vi "PathPlanner_TrajectoryState_Interpolate.vi"(9 "Time":dbl, 10 "end Val":T1={"TimeSeconds"=0.0, "VelocityMPS"=0.0, "AccerationMpsSq"=0.0, "HeadingAngularVelRadPerSec"=0.0, "PositionMeters"={"X"=0.0, "Y"=1.0}, "Heading"={"VALUE"=0.0, "COS"=1.0, "SIN"=0.0}, "TargetHolonomicRotation"={"VALUE"=0.0, "COS"=1.0, "SIN"=0.0}, "CurvatureRadPerMeter"=0.0, "PathPlannerConstraints"={"MaxVelocityMps;"=0.0, "MaxAccelerationMpsSq;"=0.0, "MaxAngularVelRadPsEc;"=0.0, "MaxAngularAccRadPSecSq"=0.0, "Exists"=FALSE, "Unlimited"=FALSE, "NominalVoltageVolts"=12.0}, "DeltaPos"=0.0, "WaypointRelPos"=0.0} {"TargetHolonomicRotation"."SIN" format="%13.4f"; "TargetHolonomicRotation"."COS" format="%13.4f"; "TargetHolonomicRotation"."VALUE" format="%13.4f"; "Heading"."SIN" format="%13.4f"; "Heading"."COS" format="%13.4f"; "Heading"."VALUE" format="%13.4f"; "PositionMeters"."Y" format="%14.3f"; "PositionMeters"."X" format="%14.3f"}, 11 "in PathPlannerState":T1={"TimeSeconds"=0.0, "VelocityMPS"=0.0, "AccerationMpsSq"=0.0, "HeadingAngularVelRadPerSec"=0.0, "PositionMeters"={"X"=0.0, "Y"=1.0}, "Heading"={"VALUE"=0.0, "COS"=1.0, "SIN"=0.0}, "TargetHolonomicRotation"={"VALUE"=0.0, "COS"=1.0, "SIN"=0.0}, "CurvatureRadPerMeter"=0.0, "PathPlannerConstraints"={"MaxVelocityMps;"=0.0, "MaxAccelerationMpsSq;"=0.0, "MaxAngularVelRadPsEc;"=0.0, "MaxAngularAccRadPSecSq"=0.0, "Exists"=FALSE, "Unlimited"=FALSE, "NominalVoltageVolts"=12.0}, "DeltaPos"=0.0, "WaypointRelPos"=0.0} {"TargetHolonomicRotation"."SIN" format="%13.4f"; "TargetHolonomicRotation"."COS" format="%13.4f"; "TargetHolonomicRotation"."VALUE" format="%13.4f"; "Heading"."SIN" format="%13.4f"; "Heading"."COS" format="%13.4f"; "Heading"."VALUE" format="%13.4f"; "PositionMeters"."Y" format="%14.3f"; "PositionMeters"."X" format="%14.3f"}) -> (3 "interpolated PathPlanner State":T1={"TimeSeconds"=0.0, "VelocityMPS"=0.0, "AccerationMpsSq"=0.0, "HeadingAngularVelRadPerSec"=0.0, "PositionMeters"={"X"=0.0, "Y"=1.0}, "Heading"={"VALUE"=0.0, "COS"=1.0, "SIN"=0.0}, "TargetHolonomicRotation"={"VALUE"=0.0, "COS"=1.0, "SIN"=0.0}, "CurvatureRadPerMeter"=0.0, "PathPlannerConstraints"={"MaxVelocityMps;"=0.0, "MaxAccelerationMpsSq;"=0.0, "MaxAngularVelRadPsEc;"=0.0, "MaxAngularAccRadPSecSq"=0.0, "Exists"=FALSE, "Unlimited"=FALSE, "NominalVoltageVolts"=12.0}, "DeltaPos"=0.0, "WaypointRelPos"=0.0} {"TargetHolonomicRotation"."SIN" format="%13.4f"; "TargetHolonomicRotation"."COS" format="%13.4f"; "TargetHolonomicRotation"."VALUE" format="%13.4f"; "Heading"."SIN" format="%13.4f"; "Heading"."COS" format="%13.4f"; "Heading"."VALUE" format="%13.4f"; "PositionMeters"."Y" format="%14.3f"; "PositionMeters"."X" format="%14.3f"})   [LabVIEW 2019, in "PathPlanner24.lvlib"]
doc: "Interpolate between this state and the given state\n \nInputs: \n - trajectoryState - cluster - this trajectory state\n - endVal - cluster - State to interpolate with\n - t - double - Interpolation factor (0.0-1.0)\n\nOutputs:\n - Interpolated state - trajectory state - interpolated state"
uses:
  PathPlanner24.lvlib
  TypeDef/PathPlannerTrajectoryState.ctl
  <vilib>/Rock Robotics/WPI/ThirdParty/JAS_Junk/TrajLib/TypeDef/TRANSLATION2D.ctl
  <vilib>/Rock Robotics/WPI/ThirdParty/JAS_Junk/TrajLib/TypeDef/ROTATION2D.ctl
  TypeDef/PathPlannerPathConstraints.ctl
  <vilib>/Rock Robotics/WPI/ThirdParty/JAS_Junk/TrajLib/Translation2d_Create.vi
  <vilib>/Rock Robotics/WPI/ThirdParty/JAS_Junk/TrajLib/MathUtil_Interpolate.vi
  <vilib>/Rock Robotics/WPI/ThirdParty/JAS_Junk/TrajLib/Translation2d_GetXY.vi
  <vilib>/Rock Robotics/WPI/ThirdParty/JAS_Junk/TrajLib/Rotation2d_Plus.vi
  <vilib>/Rock Robotics/WPI/ThirdParty/JAS_Junk/TrajLib/Rotation2d_Minus.vi
  <vilib>/Rock Robotics/WPI/ThirdParty/JAS_Junk/TrajLib/MathUtil_Clamp.vi
  <vilib>/Rock Robotics/WPI/ThirdParty/JAS_Junk/TrajLib/Rotation2d_Times.vi
  <vilib>/Rock Robotics/WPI/ThirdParty/JAS_Junk/TrajLib/Rotation2d_RotateBy.vi
  <vilib>/Rock Robotics/WPI/ThirdParty/JAS_Junk/TrajLib/Rotation2d_UnaryMinus.vi
  <vilib>/Rock Robotics/WPI/ThirdParty/JAS_Junk/TrajLib/Rotation2d_CreateAngle.vi
  <vilib>/Rock Robotics/WPI/ThirdParty/JAS_Junk/TrajLib/Rotation2d_CreateXY.vi
  <vilib>/Rock Robotics/WPI/ThirdParty/JAS_Junk/TrajLib/Util_CalcDist.vi
  <vilib>/Rock Robotics/WPI/ThirdParty/JAS_Junk/TrajLib/Trajectory_Library.lvlib
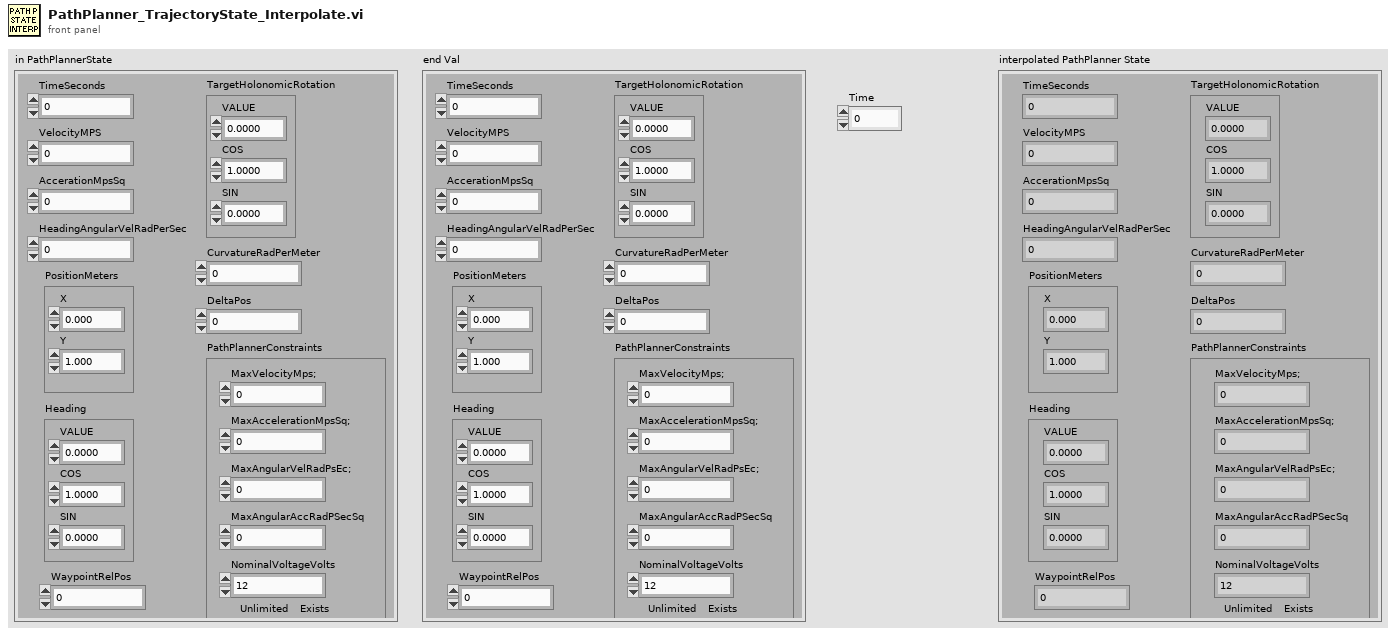
[diagram p1: front panel]
types:
  T1 = typedef "PathPlanner24.lvlib/PathPlannerTrajectoryState.ctl" = cluster{"TimeSeconds":dbl, "VelocityMPS":dbl, "AccerationMpsSq":dbl, "HeadingAngularVelRadPerSec":dbl, "PositionMeters":T2, "Heading":T3, "TargetHolonomicRotation":T3, "CurvatureRadPerMeter":dbl, "PathPlannerConstraints":T4, "DeltaPos":dbl, "WaypointRelPos":dbl}
  T2 = typedef "Trajectory_Library.lvlib/TRANSLATION2D.ctl" = cluster{"X":dbl, "Y":dbl}
  T3 = typedef "Trajectory_Library.lvlib/ROTATION2D.ctl" = cluster{"VALUE":dbl, "COS":dbl, "SIN":dbl}
  T4 = typedef "PathPlanner24.lvlib/PathPlannerPathConstraints.ctl" = cluster{"MaxVelocityMps;":dbl, "MaxAccelerationMpsSq;":dbl, "MaxAngularVelRadPsEc;":dbl, "MaxAngularAccRadPSecSq":dbl, "Exists":bool, "Unlimited":bool, "NominalVoltageVolts":dbl}
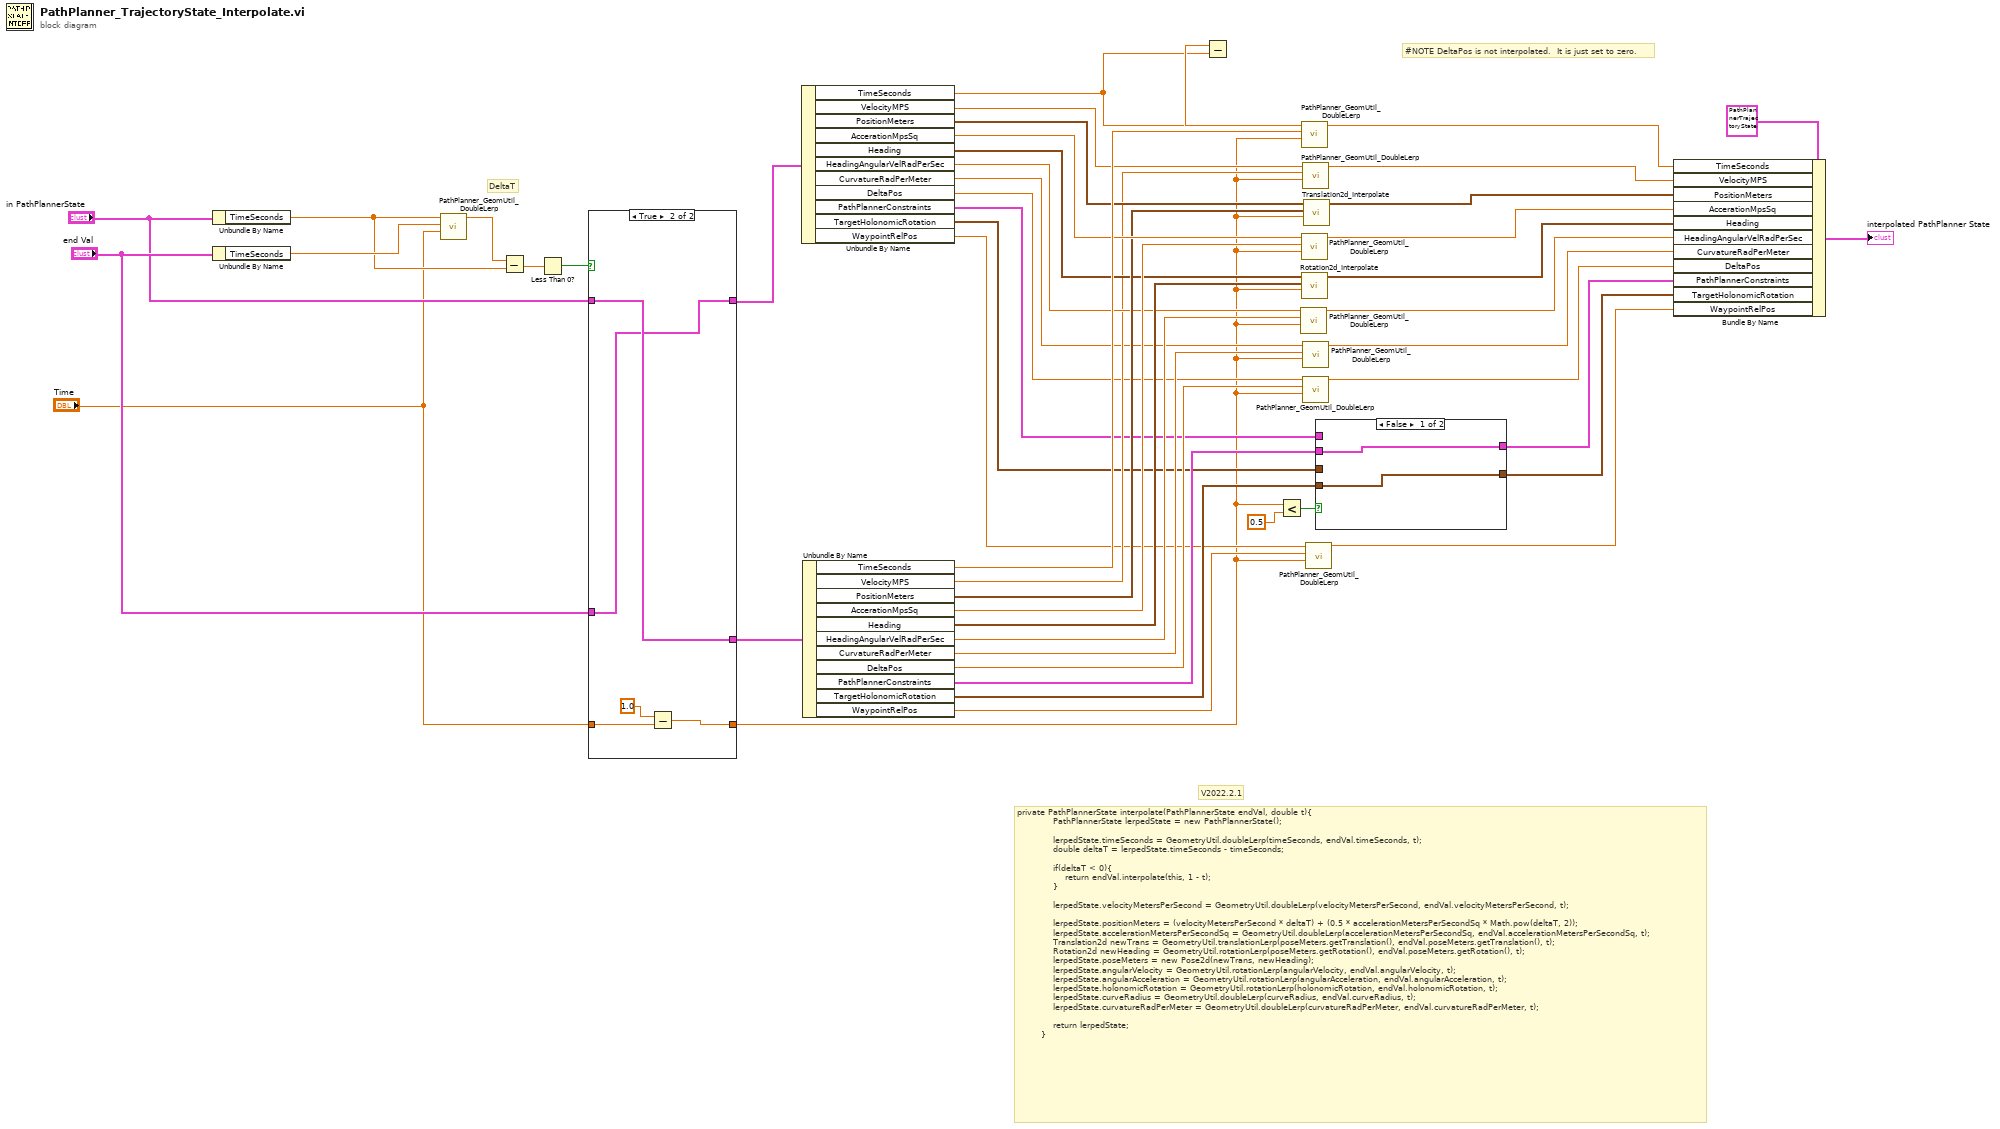
[diagram p0: block diagram]
diagram:
  # "DeltaT"
  # "V2022.2.1"
  # "private PathPlannerState interpolate(PathPlannerState endVal, double t){\n            PathPlannerState lerpedState = new PathPlannerState();\n\n            lerpedState.timeSeconds = GeometryUtil.doubleLerp(timeSeconds, endVal.timeSeconds, t);\n            double deltaT = lerpedState.timeSeconds - timeSeconds;\n\n            if(deltaT < 0){\n                return endVal.interpolate(this, 1 - t);\n            }\n\n            lerpedState.velocityMetersPerSecond = GeometryUtil.doubleLerp(velocityMetersPerSecond, endVal.velocityMetersPerSecond, t);\n\n            lerpedState.positionMeters = (velocityMetersPerSecond * deltaT) + (0.5 * accelerationMetersPerSecondSq * Math.pow(deltaT, 2));\n            lerpedState.accelerationMetersPerSecondSq = GeometryUtil.doubleLerp(accelerationMetersPerSecondSq, endVal.accelerationMetersPerSecondSq, t);\n            Translation2d newTrans = GeometryUtil.translationLerp(poseMeters.getTranslation(), endVal.poseMeters.getTranslation(), t);\n            Rotation2d newHeading = GeometryUtil.rotationLerp(poseMeters.getRotation(), endVal.poseMeters.getRotation(), t);\n            lerpedState.poseMeters = new Pose2d(newTrans, newHeading);\n            lerpedState.angularVelocity = GeometryUtil.rotationLerp(angularVelocity, endVal.angularVelocity, t);\n            lerpedState.angularAcceleration = GeometryUtil.rotationLerp(angularAcceleration, endVal.angularAcceleration, t);\n            lerpedState.holonomicRotation = GeometryUtil.rotationLerp(holonomicRotation, endVal.holonomicRotation, t);\n            lerpedState.curveRadius = GeometryUtil.doubleLerp(curveRadius, endVal.curveRadius, t);\n            lerpedState.curvatureRadPerMeter = GeometryUtil.doubleLerp(curvatureRadPerMeter, endVal.curvatureRadPerMeter, t);\n\n            return lerpedState;\n        }"
  # "#NOTE DeltaPos is not interpolated.  It is just set to zero."
  n1 = Unbundle By Name("in PathPlannerState") -> ("TimeSeconds"=w44:dbl)
  n2 = Unbundle By Name("end Val") -> ("TimeSeconds"=w46:dbl)
  n3 = call "PathPlanner_GeomUtil_DoubleLerp.vi"("T"="Time", "EndVal"=w46, "StartVal"=w44) -> ("Lerp"=w45:dbl)  [unwired: 8 in]
  n4 = Subtract(x=w45, y=w44) -> (x-y=w43:dbl)
  n5 = Less Than 0?(x=w43) -> (x < 0?=w42:bool)
  n6 = case shown="True" w42 {
    tunnel: "end Val" -> [w51 w55]
    tunnel: [w51 w56] -> w37
    tunnel: "in PathPlannerState" -> [w50 w56]
    tunnel: [w50 w55] -> w38
    tunnel: [w49 w52] -> w2
    tunnel: "Time" -> [w49 w53]
    frame False {
    }
    frame True {
      n7 = Subtract(x=1.0, y=w53) -> (x-y=w52:dbl)
    }
  }
  n8 = Unbundle By Name(w38) -> ("TimeSeconds"=w34:dbl, "VelocityMPS"=w30:dbl, "PositionMeters"=w29:T2, "AccerationMpsSq"=w33:dbl, "Heading"=w25:T3, "HeadingAngularVelRadPerSec"=w22:dbl, "CurvatureRadPerMeter"=w18:dbl, "DeltaPos"=w15:dbl, "PathPlannerConstraints"=w10:T4, "TargetHolonomicRotation"=w7:T3, "WaypointRelPos"=w4:dbl)
  n9 = Unbundle By Name(w37) -> ("TimeSeconds"=w36:dbl, "VelocityMPS"=w21:dbl, "PositionMeters"=w27:T2, "AccerationMpsSq"=w28:dbl, "Heading"=w24:T3, "HeadingAngularVelRadPerSec"=w20:dbl, "CurvatureRadPerMeter"=w17:dbl, "DeltaPos"=w14:dbl, "PathPlannerConstraints"=w9:T4, "TargetHolonomicRotation"=w6:T3, "WaypointRelPos"=w3:dbl)
  n10 = Less?(x=w2, y=0.5) -> (x < y?=w11:bool)
  n11 = call "PathPlanner_GeomUtil_DoubleLerp.vi"("T"=w2, "EndVal"=w20, "StartVal"=w22) -> ("Lerp"=w19:dbl)  [unwired: 8 in]
  n12 = call "PathPlanner_GeomUtil_DoubleLerp.vi"("T"=w2, "EndVal"=w36, "StartVal"=w34) -> ("Lerp"=w35:dbl)  [unwired: 8 in]
  n13 = Subtract(x=w35, y=w34) -> ()  [unwired: 1 out]
  n14 = call "PathPlanner_GeomUtil_DoubleLerp.vi"("T"=w2, "EndVal"=w28, "StartVal"=w33) -> ("Lerp"=w32:dbl)  [unwired: 8 in]
  n15 = call <vilib>:"Rotation2d_Interpolate.vi"("T"=w2, "EncValue ROTATION"=w24, "in ROTATION"=w25) -> ("Interpolated ROTATION"=w23:T3)  [unwired: 8 in]
  n16 = call "PathPlanner_GeomUtil_DoubleLerp.vi"("T"=w2, "EndVal"=w21, "StartVal"=w30) -> ("Lerp"=w31:dbl)  [unwired: 8 in]
  n17 = call "PathPlanner_GeomUtil_DoubleLerp.vi"("T"=w2, "EndVal"=w17, "StartVal"=w18) -> ("Lerp"=w16:dbl)  [unwired: 8 in]
  n18 = call "PathPlanner_GeomUtil_DoubleLerp.vi"("T"=w2, "EndVal"=w14, "StartVal"=w15) -> ("Lerp"=w13:dbl)  [unwired: 8 in]
  n19 = call <vilib>:"Translation2d_Interpolate.vi"("T"=w2, "other Translation"=w27, "In Translation"=w29) -> ("Interpolated Translation"=w26:T2)  [unwired: 8 in]
  n20 = call "PathPlanner_GeomUtil_DoubleLerp.vi"("T"=w2, "EndVal"=w3, "StartVal"=w4) -> ("Lerp"=w1:dbl)  [unwired: 8 in]
  n21 = case shown="False" w11 {
    tunnel: w10 -> [_ w60]
    tunnel: w9 -> [w58 _]
    tunnel: [w58 w60] -> w8
    tunnel: w7 -> [_ w59]
    tunnel: w6 -> [w57 _]
    tunnel: [w57 w59] -> w5
    frame False {
    }
    frame True {
    }
  }
  n22 = Bundle By Name(cluster=T1 {"TimeSeconds"=0.0, "VelocityMPS"=0.0, "AccerationMpsSq"=0.0, "HeadingAngularVelRadPerSec"=0.0, "PositionMeters"={"X"=0.0, "Y"=1.0}, "Heading"={"VALUE"=0.0, "COS"=1.0, "SIN"=0.0}, "TargetHolonomicRotation"={"VALUE"=0.0, "COS"=1.0, "SIN"=0.0}, "CurvatureRadPerMeter"=0.0, "PathPlannerConstraints"={"MaxVelocityMps;"=0.0, "MaxAccelerationMpsSq;"=0.0, "MaxAngularVelRadPsEc;"=0.0, "MaxAngularAccRadPSecSq"=0.0, "Exists"=FALSE, "Unlimited"=FALSE, "NominalVoltageVolts"=12.0}, "DeltaPos"=0.0, "WaypointRelPos"=0.0} ("PathPlannerState"), "TimeSeconds"=w35, "VelocityMPS"=w31, "PositionMeters"=w26, "AccerationMpsSq"=w32, "Heading"=w23, "HeadingAngularVelRadPerSec"=w19, "CurvatureRadPerMeter"=w16, "DeltaPos"=w13, "PathPlannerConstraints"=w8, "TargetHolonomicRotation"=w5, "WaypointRelPos"=w1) -> (→"interpolated PathPlanner State":T1)
